vi "Timing_Save.vi"(0 "File name":string="timing.csv", 5 "Ms":i32[](array[numeric]), 7 "Tick":i32[](array[numeric]), 11 "error in":errorcluster) -> (15 "error out":errorcluster)   [LabVIEW 2020, in "GH_App.lvlib"]
doc: "Writes a timing log to Resourcesòta\\<File name>: one line \"ms;tick\" per entry (header line first). Entries with ms = 0 were never filled and are left out."
uses:
  GH_App.lvlib
  Level/GH_Level.lvlib
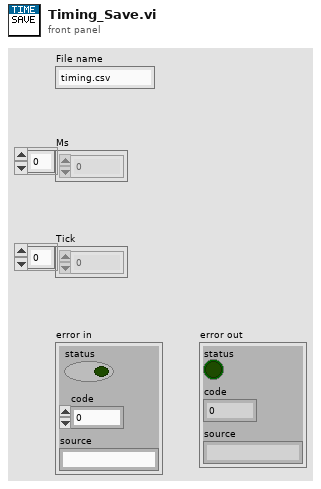
[diagram p1: front panel]
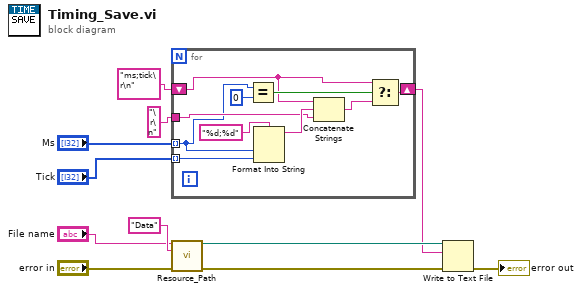
[diagram p0: block diagram]
diagram:
  n1 = for {
    tunnel: "Ms" -> [w12] mode=indexing
    tunnel: "Tick" -> [w13] mode=indexing
    tunnel: "\r\n" -> [w14]
    shift-right: [w16] -> w7
    shift-left: "ms;tick\r\n" ("Header") -> [w15]
    n2 = Equal?(x=w12, y=0) -> (x = y?=w21:bool)
    n3 = Format Into String(format string="%d;%d", w12, w13) -> (resulting string=w18:string)  [unwired: 2 in, 1 out]
    n4 = Concatenate Strings(w15, w18, w14) -> (w19:string)
    n5 = Select(t=w15, s=w21, f=w19) -> (s? t:f=w16:string)
  }
  n6 = call "Resource_Path.vi"("File name"="File name", "Subfolder"="Data", "error in"="error in") -> ("Path"=w9:path, "error out"=w10:errorcluster)  [unwired: 11 in]
  n7 = Write to Text File(file (use dialog)=w9, text=w7, error in=w10) -> (error out=→"error out":errorcluster)  [unwired: 1 in, 2 out]
